vi "TCP Message Interpreter.vi"(8 "error in (no error)":errorcluster, 9 "Data":variant, 10 "Message":string, 11 "Guardian in":refnum<class "Guardian.lvclass">) -> (0 "error out":errorcluster, 3 "Guardian out":refnum<class "Guardian.lvclass">)   [LabVIEW 2020, in "TALOS.lvlib" / "Guardian.lvlib" / "Guardian.lvclass"]
doc: "Use this VI to send a message to the Guardian, from the outside (i.e. from a uService). For internal messages, use the Actor Framework messages system."
uses:
  Guardian.lvclass
  C:/LabVIEW Code/TALOS/builds/Actor Framework PPL/Actor Framework.lvlibp/1abvi3w/vi.lib/ActorFramework/Actor/Actor.lvclass
  C:/LabVIEW Code/TALOS/talos/Ancestor/Ancestor/Ancestor.lvclass
  Ancestor/Ancestor/Ancestor.lvclass/Ancestor.ctl
  Guardian Messages/Ready to launch Msg/Ready to launch Msg.lvclass/Ready to launch Msg.ctl
  Father of all uServices/Father of all uServices/Event Handler Items.ctl
  Guardian.lvclass/Guardian.ctl
  Guardian Messages/Message to uService Msg/Message to uService Msg.lvclass/Message to uService Msg.ctl
  Ancestor/Ancestor/Infinite Message Selector.ctl
  Guardian Messages/Message to Other Guardian Msg/Message to Other Guardian Msg.lvclass/Message to Other Guardian Msg.ctl
  Classes/uService List/uService List.lvclass/uService List.ctl
  Git Update Cluster.ctl
  Abort Message.ctl
  builds/Actor Framework PPL/Actor Framework.lvlibp/1abvi3w/vi.lib/ActorFramework/Message Enqueuer/Message Priority.ctl
  Guardian Messages/Raise or Lower Abort Msg/Raise or Lower Abort Msg.lvclass/Raise or Lower Abort Msg.ctl
  Run Config Data.ctl
  Ancestor/Ancestor/Read Distr uS Map ref.vi
  Ancestor/Ancestor/Write Distr uS Map ref.vi
  Ancestor/Ancestor/Read ID.vi
  Read Guardian List.vi
  Write Guardian List.vi
  FGV/Error Memory/Get Error Description.vi
  Support VIs/Get PC name.vi
  Support VIs/Get Class Name.vi
  <vilib>/Utility/error.llb/Clear Errors.vi
  Support VIs/Circus Root Path.vi
  FGV/Error Memory/Error Memory Core.vi
  <vilib>/AdvancedString/Delimited String to 1D String Array.vi
  FGV/Error Memory/Error Crt Lvl checker.vi
  FGV/Error Memory/Error Memory Core.vi/40c8088d-b597-4017-91af-faa98e00292e.vi
  FGV/Error Memory/Error Memory Core.vi/d4a3ab98-063c-4e44-b43d-fbdcfe6c2be2.vi
  Support VIs/Global Memory.vi
  <vilib>/Utility/LVClass/Get LV Class Name.vi
  Support VIs/TALOS Root path.vi
  Support VIs/Read CSV worksheet.vi
  Support VIs/Global Constants.vi
  <vilib>/Utility/error.llb/General Error Handler.vi
  builds/Actor Framework PPL/Actor Framework.lvlibp/1abvi3w/vi.lib/ActorFramework/Message Enqueuer/Enqueue.vi
  Support VIs/Error Log.vi
  <vilib>/Utility/config.llb/Open Config Data.vi
  <vilib>/Utility/config.llb/Get Section Names.vi
  <vilib>/Utility/config.llb/Get Key Names.vi
  <vilib>/Utility/config.llb/Read Key.vi
  <vilib>/Utility/config.llb/Read Key (String).vi
  <vilib>/Utility/config.llb/Close Config Data.vi
  Ancestor/Ancestor/Ancestor.lvclass
  <vilib>/Comparison/Equal/Equal Functor/Equal Functor.lvclass
  Guardian Messages/Ready to launch Msg/Ready to launch Msg.lvclass
  Guardian Messages/Message to uService Msg/Message to uService Msg.lvclass
  Guardian Messages/Message to Other Guardian Msg/Message to Other Guardian Msg.lvclass
  Classes/Distributed uService Map/Distributed uService Map.lvclass
  Classes/Guardian List/Guardian List.lvclass
  Guardian Messages/Raise or Lower Abort Msg/Raise or Lower Abort Msg.lvclass
  TALOS.lvlib
  Father of all uServices/Father of all uServices/Father of all uServices.lvclass
  builds/Actor Framework PPL/Actor Framework.lvlibp/1abvi3w/vi.lib/ActorFramework/Message Enqueuer/Message Enqueuer.lvclass
  builds/Actor Framework PPL/Actor Framework.lvlibp/1abvi3w/vi.lib/ActorFramework/Actor/Actor.lvclass
  Im alive message.ctl
  Classes/uService List/uService List.lvclass
  Classes/Error Filter/Error Filter.lvclass
  FGV/Error Memory/Error Memory.lvlib
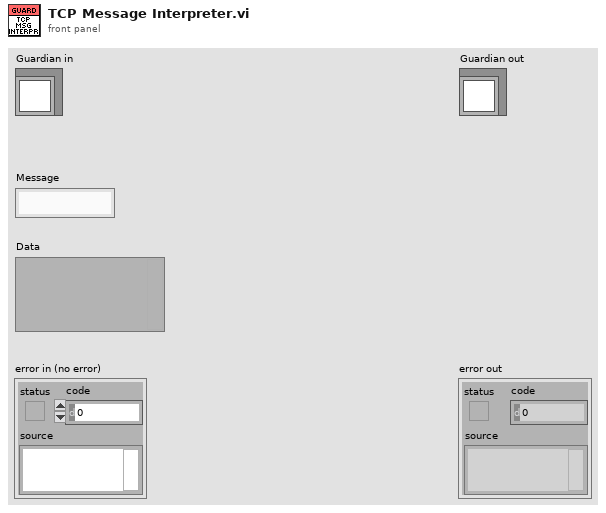
[diagram p1: front panel]
types:
  T1 = typedef "TALOS.lvlib/Father of all uServices.lvlib/Father of all uServices.lvclass/Event Handler Items.ctl" = enum16{"Button Pressed", "Message", "Ready to launch?", "Safe Mode", "Start RUN", "Stop RUN"}
  T2 = typedef "TALOS.lvlib/Ancestor.lvlib/Ancestor.lvclass/Infinite Message Selector.ctl" = enum16{"Start", "Stop", "Check", "Flush (Stop all)", "Init"}
  T3 = typedef "TALOS.lvlib/Guardian.lvlib/Guardian.lvclass/Im alive message.ctl" = cluster{"ID":string, "Time":timestamp, "Abort":bool, "Bearer":bool}
  T4 = typedef "TALOS.lvlib/Guardian.lvlib/Guardian.lvclass/Git Update Cluster.ctl" = cluster{"branch name":string, "include critical PCs":bool, "update from git":bool}
  T5 = typedef "Actor Framework.lvlibp/Message Enqueuer.lvclass/Message Priority.ctl" = enum16{"Low", "Normal", "High"}
  T6 = typedef "TALOS.lvlib/Guardian.lvlib/Guardian.lvclass/Abort Message.ctl" = cluster{"4b0rt":bool, "Sender":string}
  T7 = typedef "TALOS.lvlib/Guardian.lvlib/Guardian.lvclass/Run Config Data.ctl" = cluster{"Name":string, "uS List":string[]}
  T8 = cluster{"Accessors:ID":string, "All IDs":string[]}
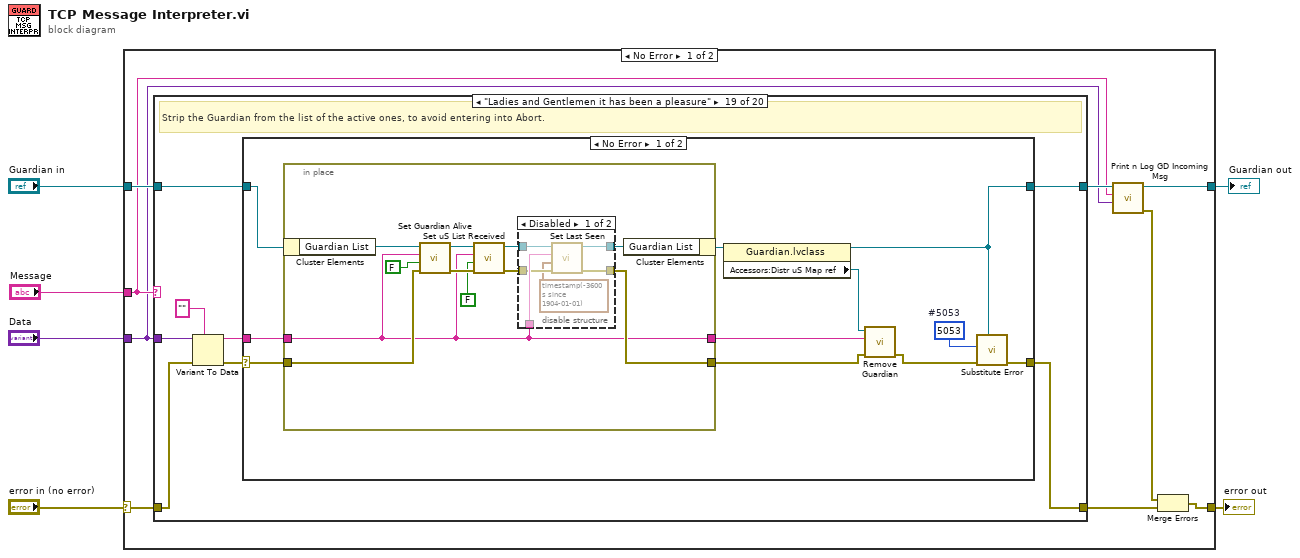
[diagram p0: block diagram]
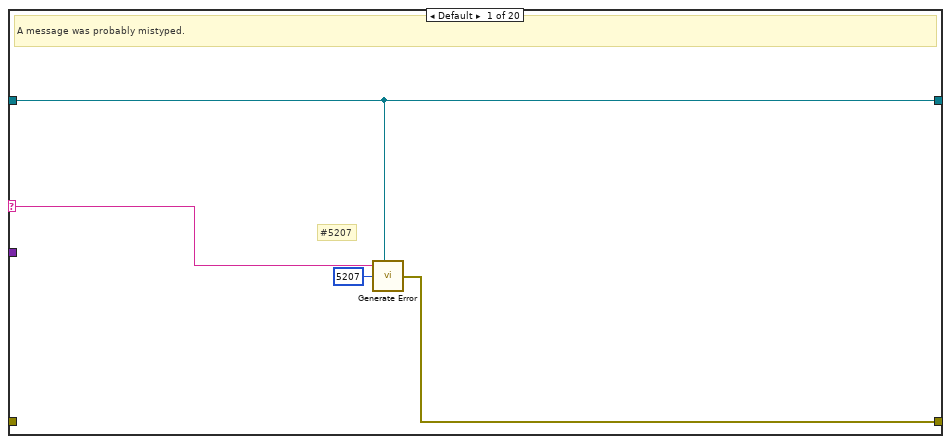
[diagram p2: hidden frame]
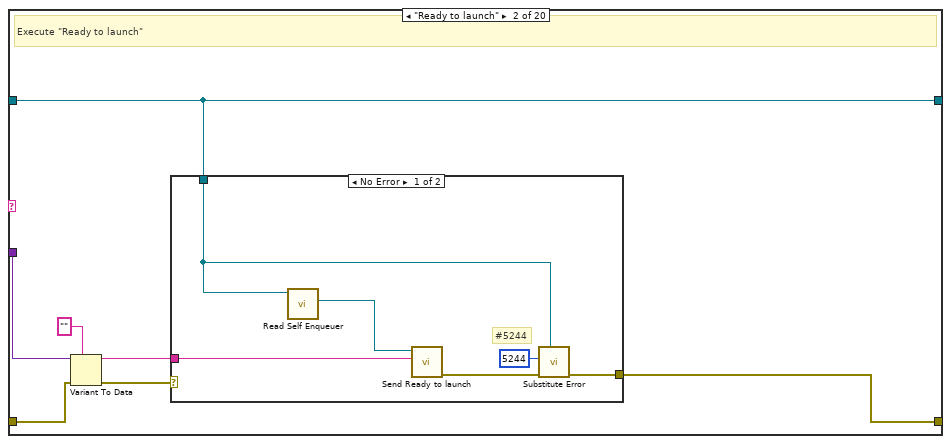
[diagram p3: hidden frame]
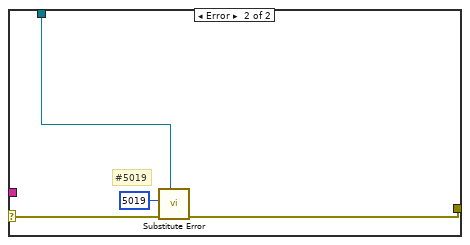
[diagram p4: hidden frame]
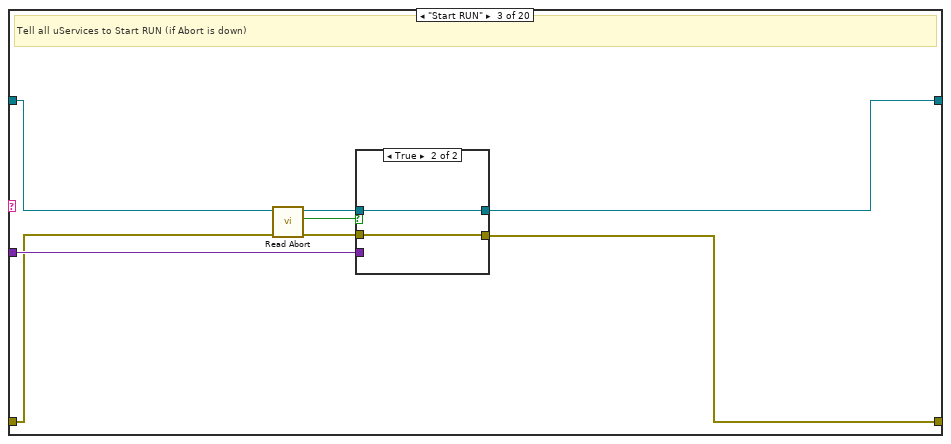
[diagram p5: hidden frame]
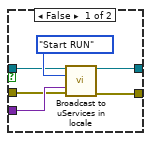
[diagram p6: hidden frame]
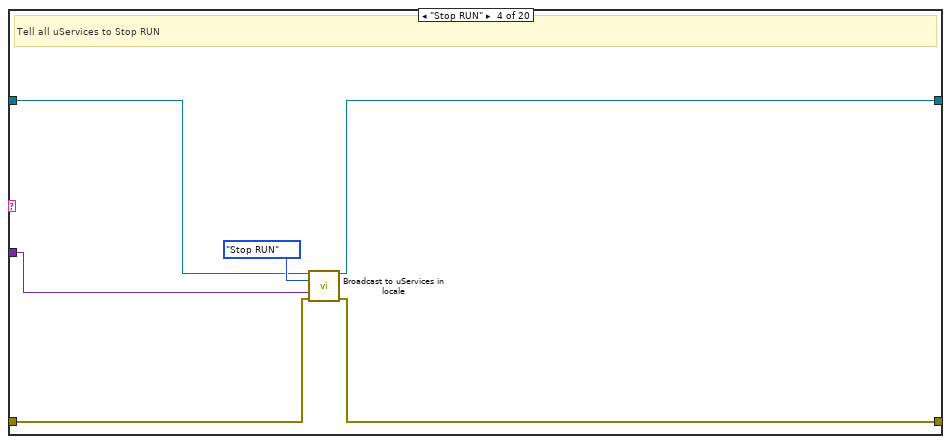
[diagram p7: hidden frame]
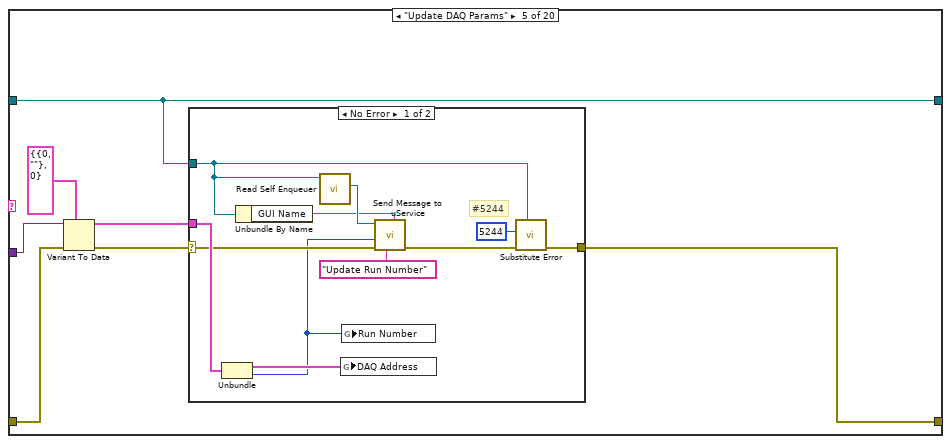
[diagram p8: hidden frame]
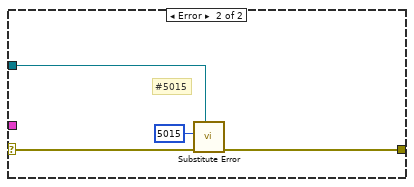
[diagram p9: hidden frame]
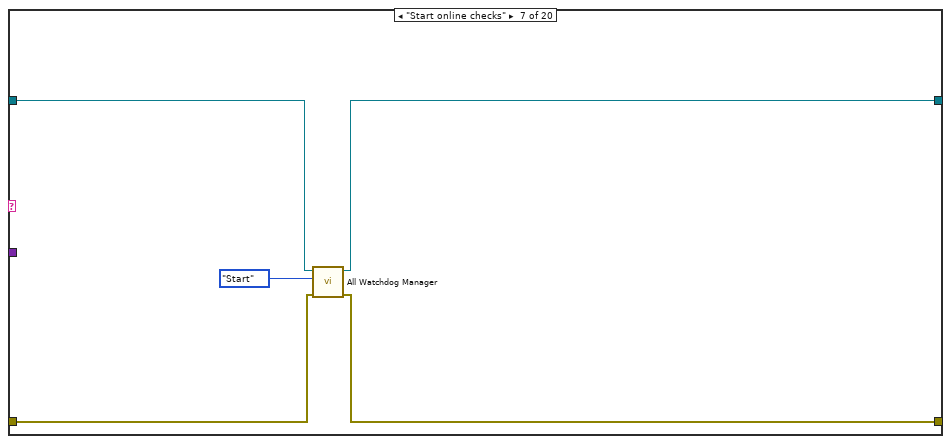
[diagram p11: hidden frame]
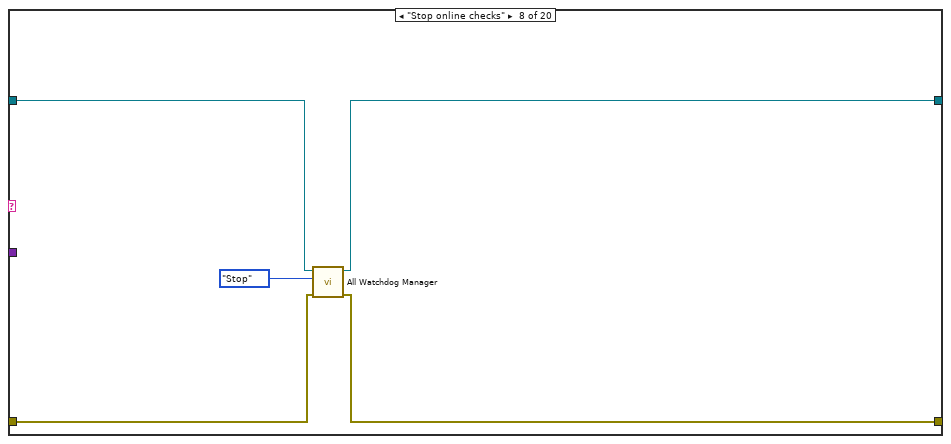
[diagram p12: hidden frame]
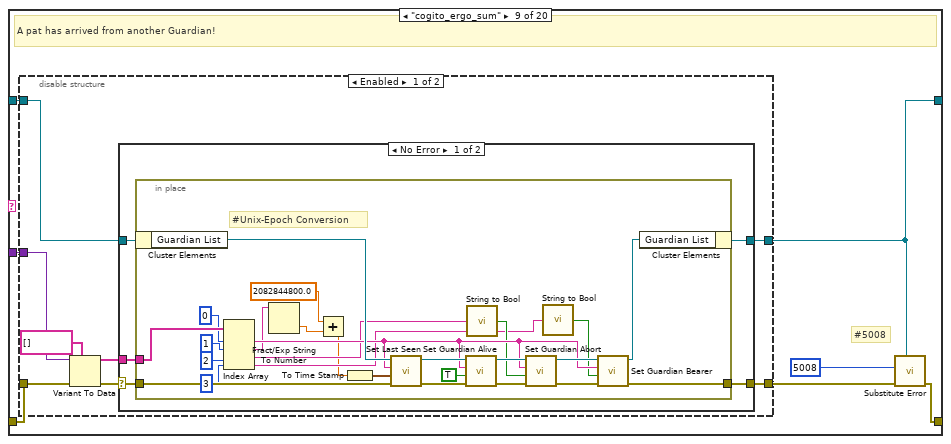
[diagram p13: hidden frame]
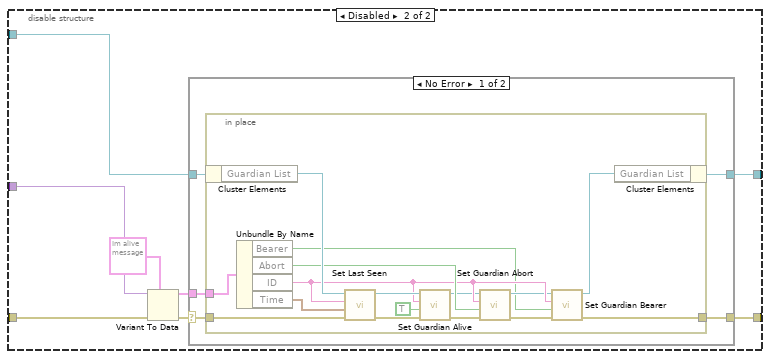
[diagram p15: hidden frame]
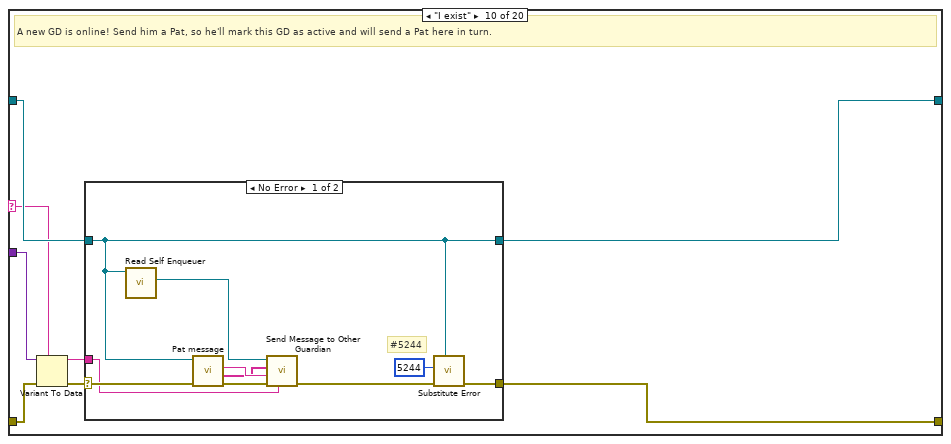
[diagram p17: hidden frame]
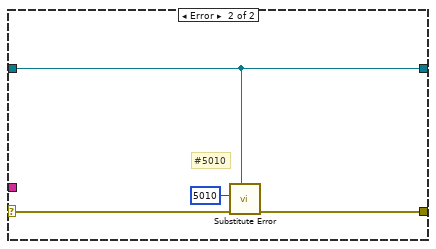
[diagram p18: hidden frame]
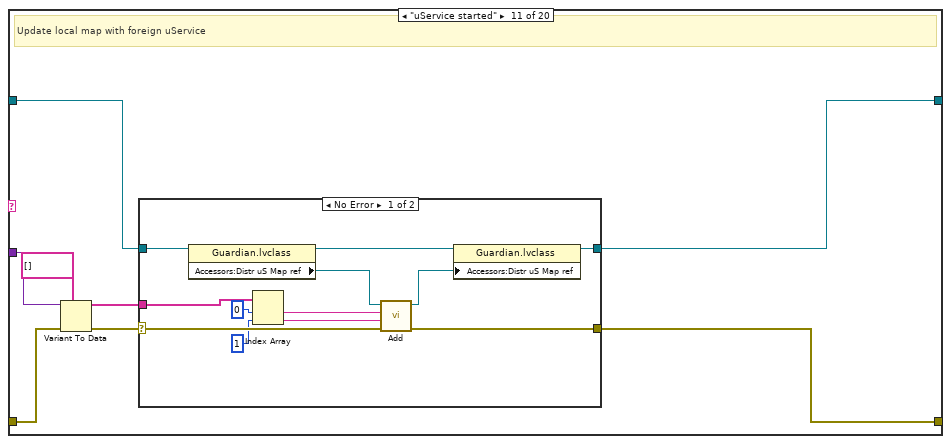
[diagram p19: hidden frame]
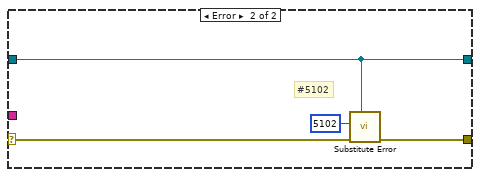
[diagram p20: hidden frame]
diagram:
  n1 = case shown="No Error" "error in (no error)" {
    selector: "error in (no error)" -> [w14 w456]
    tunnel: [w13 w456] -> w6
    tunnel: "Guardian in" -> [w12 w455]
    tunnel: [w10 w455] -> w3
    tunnel: "Data" -> [w8 _]
    tunnel: "Message" -> [w9 _]
    frame No Error {
      n2 = case shown="\"Ladies and Gentlemen it has been a pleasure\"" w9 {
        selector: w9 -> [w17 _ _ _ _ _ _ _ _ w173 _ _ _ _ _ w317 _ _ _ w416]
        tunnel: [w18 w25 w43 w56 w60 w81 w84 w89 w94 w172 w194 w218 w242 w271 w303 w311 w328 w355 w373 w418] -> w15
        tunnel: w8 -> [_ w24 w42 w53 w65 _ _ _ w99 w179 w199 w223 w247 w275 _ w315 w322 w367 w380 w426]
        tunnel: w12 -> [w16 w26 w41 w54 w61 w82 w87 w92 w97 w175 w201 w225 w249 w277 w309 w310 w327 w356 w375 w421]
        tunnel: [w16 w26 w44 w57 w61 w82 w86 w91 w95 w174 w200 w224 w248 w276 w309 w310 w325 w356 w374 w417] -> w11
        tunnel: w14 -> [_ w23 w39 w55 w59 w81 w83 w88 w98 w178 w198 w222 w246 w274 w308 w314 w329 w366 w379 w425]
        frame Default {
          # "#5207"
          # "A message was probably mistyped."
          n3 = call "Generate Error.vi"("Optional String"=w17, "Class"=w16, "Error Code"=5207) -> ("error out"=w18:errorcluster)  [unwired: 4 in]
        }
        frame "Ready to launch" {
          # "Execute \"Ready to launch\""
          n4 = Variant To Data(error in=w23, type="", Variant=w24) -> (data=w20:string, error out=w21:errorcluster)
          n5 = case shown="No Error" w21 {
            selector: w21 -> [_ w35]
            tunnel: w26 -> [w27 w36]
            tunnel: [w28 w34] -> w25
            tunnel: w20 -> [w31 _]
            frame No Error {
              # "#5244"
              n6 = call "Read Self Enqueuer.vi"("Actor"=w27) -> ("Self Enqueuer"=w32:refnum<class "Message Enqueuer.lvclass">)  [unwired: 10 in]
              n7 = call "Send Ready to launch.vi"("GUID"=w31, "Message Enqueuer"=w32) -> ("error out"=w29:errorcluster)  [unwired: 8 in, 1 out]
              n8 = call "Substitute Error.vi"("LabVIEW Object"=w27, "error in (no error)"=w29, "Error Code"=5244) -> ("error out"=w28:errorcluster)  [unwired: 8 in]
            }
            frame Error {
              # "#5019"
              n9 = call "Substitute Error.vi"("LabVIEW Object"=w36, "error in (no error)"=w35, "Error Code"=5019) -> ("error out"=w34:errorcluster)  [unwired: 8 in]
            }
          }
        }
        frame "Start RUN" {
          # "Tell all uServices to Start RUN (if Abort is down)"
          n10 = call "Read Abort.vi"("error in (no error)"=w39, "Guardian in"=w41) -> ("error out"=w38:errorcluster, "Abort"=w37:bool, "Guardian out"=w40:refnum<class "Guardian.lvclass">)  [unwired: 7 in]
          n11 = case shown="True" w37 {
            tunnel: [w49 w52] -> w44
            tunnel: [w48 w51] -> w43
            tunnel: w42 -> [w47 _]
            tunnel: w40 -> [w46 w52]
            tunnel: w38 -> [w45 w51]
            frame False {
              n12 = call "Broadcast to uServices in locale.vi"("Guardian in"=w46, "Event type"=Event_Handler_Items."Start RUN", "Data"=w47, "error in (no error)"=w45) -> ("Guardian out"=w49:refnum<class "Guardian.lvclass">, "error out"=w48:errorcluster)  [unwired: 10 in]
            }
            frame True {
            }
          }
        }
        frame "Stop RUN" {
          # "Tell all uServices to Stop RUN"
          n13 = call "Broadcast to uServices in locale.vi"("Guardian in"=w54, "Event type"=Event_Handler_Items."Stop RUN", "Data"=w53, "error in (no error)"=w55) -> ("Guardian out"=w57:refnum<class "Guardian.lvclass">, "error out"=w56:errorcluster)  [unwired: 10 in]
        }
        frame "Update DAQ Params" {
          n14 = Variant To Data(error in=w59, type=cluster{cluster{u16, string}, i32} {{0, ""}, 0}, Variant=w65) -> (data=w63:cluster{cluster{u16, string}, i32}, error out=w62:errorcluster)
          n15 = case shown="No Error" w62 {
            selector: w62 -> [w73 w80]
            tunnel: w63 -> [w74 _]
            tunnel: w61 -> [w67 w78]
            tunnel: [w66 w79] -> w60
            frame No Error {
              # "#5244"
              n16 = Unbundle(w74) -> (w71:cluster{u16, string}, w70:i32)
              n17 = Unbundle By Name(w67) -> ("GUI Name"=w75:string)
              n18 = call "Read Self Enqueuer.vi"("Actor"=w67) -> ("Self Enqueuer"=w76:refnum<class "Message Enqueuer.lvclass">)  [unwired: 10 in]
              n19 = global write "Global Memory.vi" "DAQ Address"(w71) -> ()
              n20 = global write "Global Memory.vi" "Run Number"(w70) -> ()
              n21 = call "Send Message to uService.vi"("uService ID"=w75, "Message"="Update Run Number", "error in (no error)"=w73, "Data"=w70, "Message Enqueuer"=w76) -> ("error out"=w68:errorcluster)  [unwired: 5 in, 1 out]
              n22 = call "Substitute Error.vi"("LabVIEW Object"=w67, "error in (no error)"=w68, "Error Code"=5244) -> ("error out"=w66:errorcluster)  [unwired: 8 in]
            }
            frame Error {
              # "#5015"
              n23 = call "Substitute Error.vi"("LabVIEW Object"=w78, "error in (no error)"=w80, "Error Code"=5015) -> ("error out"=w79:errorcluster)  [unwired: 8 in]
            }
          }
        }
        frame "Text Message" {
          # "For testing purpouses"
        }
        frame "Start online checks" {
          n24 = call "All Watchdog Manager.vi"("error in (no error)"=w83, "Infinite Message Selector"=Infinite_Message_Selector."Start", "Guardian in"=w87) -> ("error out"=w84:errorcluster, "Guardian out"=w86:refnum<class "Guardian.lvclass">)  [unwired: 6 in, 1 out]
        }
        frame "Stop online checks" {
          n25 = call "All Watchdog Manager.vi"("error in (no error)"=w88, "Infinite Message Selector"=Infinite_Message_Selector."Stop", "Guardian in"=w92) -> ("error out"=w89:errorcluster, "Guardian out"=w91:refnum<class "Guardian.lvclass">)  [unwired: 6 in, 1 out]
        }
        frame "cogito_ergo_sum" {
          # "#5008"
          # "A pat has arrived from another Guardian!"
          n26 = disable-structure shown="Enabled" {
            disable-tunnel: w99 -> [w107 w148]
            disable-tunnel: w98 -> [w106 w146]
            disable-tunnel: w97 -> [w103 w143]
            disable-tunnel: [w102 w142] -> w96
            disable-tunnel: [w101 w141] -> w95
            frame Enabled {
              n27 = Variant To Data(error in=w106, type=string[] [], Variant=w107) -> (data=w105:string[], error out=w104:errorcluster)
              n28 = case shown="No Error" w104 {
                selector: w104 -> [w109 w139]
                tunnel: w105 -> [w110 _]
                tunnel: w103 -> [w112 w140]
                tunnel: [w111 w140] -> w101
                tunnel: [w108 w139] -> w102
                frame No Error {
                  n29 = in-place {
                    in-place-border: w110 -> [w127]
                    in-place-border: w109 -> [w137]
                    in-place-border: [w129] -> w108
                    # "#Unix-Epoch Conversion"
                    n30 = in-place-cluster #1(w112) -> ("Guardian List"=w138:refnum<class "Guardian List.lvclass">)
                    n31 = Index Array(array=w127, index #1=0 ("index"), index #2=1 ("index"), index #3=2 ("index"), index #4=3 ("index")) -> (element #1=w122:string, element #2=w117:string, element #3=w121:string, element #4=w119:string)
                    n32 = Fract/Exp String To Number(string=w117) -> (number=w116:dbl)  [unwired: 3 in, 1 out]
                    n33 = Add(x=2082844800.0, y=w116) -> (x+y=w114:dbl)
                    n34 = To Time Stamp(1:w114) -> (0:w113:timestamp)
                    n35 = call-dynamic "Set Last Seen.vi"("error in (no error)"=w137, "Last Seen"=w113, "ID"=w122, "Guardian List in"=w138) -> ("error out"=w135:errorcluster, "Guardian List out"=w136:refnum<class "Guardian List.lvclass">)  [unwired: 6 in]
                    n36 = call-dynamic "Set Guardian Alive.vi"("error in (no error)"=w135, "Alive"=TRUE, "ID"=w122, "Guardian List in"=w136) -> ("error out"=w133:errorcluster, "Guardian List out"=w128:refnum<class "Guardian List.lvclass">)  [unwired: 6 in]
                    n37 = call "String to Bool.vi"("String"=w121) -> ("Boolean"=w120:bool)
                    n38 = call-dynamic "Set Guardian Abort.vi"("error in (no error)"=w133, "Abort"=w120, "ID"=w122, "Guardian List in"=w128) -> ("error out"=w132:errorcluster, "Guardian List out"=w131:refnum<class "Guardian List.lvclass">)  [unwired: 6 in]
                    n39 = call "String to Bool.vi"("String"=w119) -> ("Boolean"=w118:bool)
                    n40 = call-dynamic "Set Guardian Bearer.vi"("error in (no error)"=w132, "Bearer"=w118, "ID"=w122, "Guardian List in"=w131) -> ("error out"=w129:errorcluster, "Guardian List out"=w130:refnum<class "Guardian List.lvclass">)  [unwired: 6 in]
                    n41 = in-place-cluster #1("Guardian List"=w130) -> (w111:refnum<class "Guardian.lvclass">)
                  }
                }
                frame Error {
                }
              }
            }
            frame Disabled {
              n42 = Variant To Data(error in=w146, type=T3 {"ID"="", "Time"=timestamp(0 s since 1904-01-01), "Abort"=FALSE, "Bearer"=FALSE} ("cluster"), Variant=w148) -> (data=w145:T3, error out=w144:errorcluster)
              n43 = case shown="No Error" w144 {
                selector: w144 -> [w150 w170]
                tunnel: w145 -> [w151 _]
                tunnel: w143 -> [w153 w171]
                tunnel: [w152 w171] -> w141
                tunnel: [w149 w170] -> w142
                frame No Error {
                  n44 = in-place {
                    in-place-border: w151 -> [w168]
                    in-place-border: w150 -> [w166]
                    in-place-border: [w155] -> w149
                    n45 = in-place-cluster #2(w153) -> ("Guardian List"=w169:refnum<class "Guardian List.lvclass">)
                    n46 = Unbundle By Name(w168) -> ("Bearer"=w157:bool, "Abort"=w160:bool, "ID"=w159:string, "Time"=w167:timestamp)
                    n47 = call-dynamic "Set Last Seen.vi"("error in (no error)"=w166, "Last Seen"=w167, "ID"=w159, "Guardian List in"=w169) -> ("error out"=w164:errorcluster, "Guardian List out"=w165:refnum<class "Guardian List.lvclass">)  [unwired: 6 in]
                    n48 = call-dynamic "Set Guardian Alive.vi"("error in (no error)"=w164, "Alive"=TRUE, "ID"=w159, "Guardian List in"=w165) -> ("error out"=w162:errorcluster, "Guardian List out"=w154:refnum<class "Guardian List.lvclass">)  [unwired: 6 in]
                    n49 = call-dynamic "Set Guardian Abort.vi"("error in (no error)"=w162, "Abort"=w160, "ID"=w159, "Guardian List in"=w154) -> ("error out"=w161:errorcluster, "Guardian List out"=w158:refnum<class "Guardian List.lvclass">)  [unwired: 6 in]
                    n50 = call-dynamic "Set Guardian Bearer.vi"("error in (no error)"=w161, "Bearer"=w157, "ID"=w159, "Guardian List in"=w158) -> ("error out"=w155:errorcluster, "Guardian List out"=w156:refnum<class "Guardian List.lvclass">)  [unwired: 6 in]
                    n51 = in-place-cluster #2("Guardian List"=w156) -> (w152:refnum<class "Guardian.lvclass">)
                  }
                }
                frame Error {
                }
              }
            }
          }
          n52 = call "Substitute Error.vi"("LabVIEW Object"=w95, "error in (no error)"=w96, "Error Code"=5008) -> ("error out"=w94:errorcluster)  [unwired: 8 in]
        }
        frame "I exist" {
          # "A new GD is online! Send him a Pat, so he'll mark this GD as active and will send a Pat here in turn."
          n53 = Variant To Data(error in=w178, type=w173, Variant=w179) -> (data=w177:string, error out=w176:errorcluster)
          n54 = case shown="No Error" w176 {
            selector: w176 -> [w188 w192]
            tunnel: w177 -> [w187 _]
            tunnel: w175 -> [w181 w193]
            tunnel: [w181 w193] -> w174
            tunnel: [w180 w190] -> w172
            frame No Error {
              # "#5244"
              n55 = call "Read Self Enqueuer.vi"("Actor"=w181) -> ("Self Enqueuer"=w189:refnum<class "Message Enqueuer.lvclass">)  [unwired: 10 in]
              n56 = call "Pat message.vi"("error in (no error)"=w188, "Guardian in"=w181) -> ("error out"=w184:errorcluster, "Data"=w185:string[], "Message name"=w186:string)  [unwired: 6 in, 1 out]
              n57 = call "Send Message to Other Guardian.vi"("Guardian ID"=w187, "error in (no error)"=w184, "Message"=w186, "Data"=w185, "Message Enqueuer"=w189) -> ("error out"=w182:errorcluster)  [unwired: 5 in, 1 out]
              n58 = call "Substitute Error.vi"("LabVIEW Object"=w181, "error in (no error)"=w182, "Error Code"=5244) -> ("error out"=w180:errorcluster)  [unwired: 8 in]
            }
            frame Error {
              # "#5010"
              n59 = call "Substitute Error.vi"("LabVIEW Object"=w193, "error in (no error)"=w192, "Error Code"=5010) -> ("error out"=w190:errorcluster)  [unwired: 8 in]
            }
          }
        }
        frame "uService started" {
          # "Update local map with foreign uService"
          n60 = Variant To Data(error in=w198, type=string[] [], Variant=w199) -> (data=w195:string[], error out=w196:errorcluster)
          n61 = case shown="No Error" w196 {
            selector: w196 -> [w213 w217]
            tunnel: w201 -> [w206 w215]
            tunnel: [w203 w215] -> w200
            tunnel: w195 -> [w211 _]
            tunnel: [w212 w214] -> w194
            frame No Error {
              n62 = property class="Guardian.lvclass"(reference=w206) -> (reference out=w204:refnum<class "Guardian.lvclass">, "Accessors:Distr uS Map ref"=w205:refnum<data-value>)  [unwired: 1 in, 1 out]
              n63 = Index Array(array=w211, index #1=0 ("index"), index #2=1 ("index")) -> (element #1=w208:string, element #2=w207:string)
              n64 = call "Add.vi"("error in (no error)"=w213, "uService"=w207, "Guardian"=w208, "Distr uS Map ref in"=w205) -> ("error out"=w212:errorcluster, "Distr uS Map ref out"=w202:refnum<data-value>)  [unwired: 5 in, 1 out]
              n65 = property class="Guardian.lvclass"(reference=w204, "Accessors:Distr uS Map ref"=w202) -> (reference out=w203:refnum<class "Guardian.lvclass">)  [unwired: 1 in, 1 out]
            }
            frame Error {
              # "#5102"
              n66 = call "Substitute Error.vi"("LabVIEW Object"=w215, "error in (no error)"=w217, "Error Code"=5102) -> ("error out"=w214:errorcluster)  [unwired: 8 in]
            }
          }
        }
        frame "uService stopped" {
          # "Update local map with foreign uService"
          n67 = Variant To Data(error in=w222, type=string[] [], Variant=w223) -> (data=w219:string[], error out=w220:errorcluster)
          n68 = case shown="No Error" w220 {
            selector: w220 -> [w236 w241]
            tunnel: w225 -> [w237 w239]
            tunnel: [w227 w239] -> w224
            tunnel: w219 -> [w234 _]
            tunnel: [w235 w238] -> w218
            frame No Error {
              n69 = property class="Guardian.lvclass"(reference=w237) -> (reference out=w228:refnum<class "Guardian.lvclass">, "Accessors:Distr uS Map ref"=w229:refnum<data-value>)  [unwired: 1 in, 1 out]
              n70 = Index Array(array=w234, index #1=0 ("index"), index #2=1 ("index")) -> (element #1=w231:string, element #2=w230:string)
              n71 = call "Remove.vi"("error in (no error)"=w236, "uService ID"=w230, "Guardian"=w231, "Distr uS Map ref in"=w229) -> ("error out"=w235:errorcluster, "Distr uS Map ref out"=w226:refnum<data-value>)  [unwired: 5 in, 1 out]
              n72 = property class="Guardian.lvclass"(reference=w228, "Accessors:Distr uS Map ref"=w226) -> (reference out=w227:refnum<class "Guardian.lvclass">)  [unwired: 1 in, 1 out]
            }
            frame Error {
              # "#5102"
              n73 = call "Substitute Error.vi"("LabVIEW Object"=w239, "error in (no error)"=w241, "Error Code"=5102) -> ("error out"=w238:errorcluster)  [unwired: 8 in]
            }
          }
        }
        frame "Get uService List" {
          # "Give to the requesting Guardian the current uService List (for initialise the distributed one)"
          n74 = Variant To Data(error in=w246, type="", Variant=w247) -> (data=w243:string, error out=w244:errorcluster)
          n75 = case shown="No Error" w244 {
            selector: w244 -> [w260 w269]
            tunnel: w249 -> [w261 w267]
            tunnel: [w250 w267] -> w248
            tunnel: w243 -> [w265 _]
            tunnel: [w251 w266] -> w242
            frame No Error {
              # "#5244"
              # "requesting GD"
              n76 = call-dynamic "Access uService List.vi"("error in (no error)"=w260, "Ancestor in"=w261) -> ("error out"=w258:errorcluster, "uService List out"=w259:refnum<class "uService List.lvclass">, "Ancestor out"=w262:refnum<class "Guardian.lvclass">)  [unwired: 7 in]
              n77 = call "Get all IDs.vi"("error in (no error)"=w258, "uService List"=w259) -> ("error out"=w257:errorcluster, "All IDs"=w255:string[])  [unwired: 7 in, 1 out]
              n78 = property class="Guardian.lvclass"(reference=w262) -> (reference out=w250:refnum<class "Guardian.lvclass">, "Accessors:ID"=w256:string)  [unwired: 1 in, 1 out]
              n79 = Bundle("Accessors:ID"=w256, "All IDs"=w255) -> (w254:T8)  [unwired: 1 in]
              n80 = call "Read Self Enqueuer.vi"("Actor"=w250) -> ("Self Enqueuer"=w264:refnum<class "Message Enqueuer.lvclass">)  [unwired: 10 in]
              n81 = call "Send Message to Other Guardian.vi"("Guardian ID"=w265, "error in (no error)"=w257, "Message"="Current uService List", "Data"=w254, "Message Enqueuer"=w264) -> ("error out"=w252:errorcluster)  [unwired: 5 in, 1 out]
              n82 = call "Substitute Error.vi"("LabVIEW Object"=w250, "error in (no error)"=w252, "Error Code"=5244) -> ("error out"=w251:errorcluster)  [unwired: 8 in]
            }
            frame Error {
              # "#5102"
              n83 = call "Substitute Error.vi"("LabVIEW Object"=w267, "error in (no error)"=w269, "Error Code"=5102) -> ("error out"=w266:errorcluster)  [unwired: 8 in]
            }
          }
        }
        frame "Current uService List" {
          # "Update Distributed uService List with the list received"
          n84 = Variant To Data(error in=w274, type=cluster{"String":string, string[]} {"String"="", []}, Variant=w275) -> (data=w272:cluster{"String":string, string[]}, error out=w273:errorcluster)
          n85 = case shown="No Error" w273 {
            selector: w273 -> [w291 w302]
            tunnel: w277 -> [w284 w300]
            tunnel: [w283 w300] -> w276
            tunnel: w272 -> [w292 _]
            tunnel: [w290 w299] -> w271
            frame No Error {
              n86 = property class="Guardian.lvclass"(reference=w284) -> (reference out=w280:refnum<class "Guardian.lvclass">, "Accessors:Distr uS Map ref"=w279:refnum<data-value>, "Accessors:Guardian List"=w278:refnum<class "Guardian List.lvclass">)  [unwired: 1 in, 1 out]
              n87 = Unbundle(w292) -> ("String"=w287:string, w289:string[])
              n88 = for {
                shift-right: [w294] -> w282
                shift-left: w279 -> [w293]
                tunnel: w287 -> [w298]
                tunnel: w289 -> [w297] mode=indexing
                shift-right: [w295] -> w288
                shift-left: w291 -> [w296]
                n89 = call "Add.vi"("error in (no error)"=w296, "uService"=w297, "Guardian"=w298, "Distr uS Map ref in"=w293) -> ("error out"=w295:errorcluster, "Distr uS Map ref out"=w294:refnum<data-value>)  [unwired: 5 in, 1 out]
              }
              n90 = call-dynamic "Set uS List Received.vi"("uS List Received"=TRUE, "ID"=w287, "Guardian List in"=w278) -> ("error out"=w286:errorcluster, "Guardian List out"=w281:refnum<class "Guardian List.lvclass">)  [unwired: 7 in]
              n91 = Merge Errors(w288, w286) -> (w290:errorcluster)
              n92 = property class="Guardian.lvclass"(reference=w280, "Accessors:Distr uS Map ref"=w282, "Accessors:Guardian List"=w281) -> (reference out=w283:refnum<class "Guardian.lvclass">)  [unwired: 1 in, 1 out]
            }
            frame Error {
              # "#5102"
              n93 = call "Substitute Error.vi"("LabVIEW Object"=w300, "error in (no error)"=w302, "Error Code"=5102) -> ("error out"=w299:errorcluster)  [unwired: 8 in]
            }
          }
        }
        frame "Reload INI files" {
          w306 = TRUE ("Load")
          # "Reload the configuration files"
          n94 = call "TALOS Config Param.vi"("Load"=w306, "error in (no error)"=w308) -> ("error out"=w307:errorcluster)  [unwired: 8 in, 1 out]
          n95 = call "Circus Config Param - Core.vi"("Load"=w306, "error in (no error)"=w307) -> ("error out"=w305:errorcluster)  [unwired: 8 in, 1 out]
          n96 = call "Errors Load.vi"("error in (no error)"=w305) -> ("error out"=w304:errorcluster)  [unwired: 10 in]
          n97 = call "Init.vi"("error in (no error)"=w304) -> ("error out"=w303:errorcluster)  [unwired: 10 in]
        }
        frame "Change Run LED color", "Reset Run LED", "Run Stopped with Errors", "Update Error Listbox", "Update Kasli Log", "Update Run Status" {
          # "#5244"
          n98 = Unbundle By Name(w310) -> ("GUI Name"=w318:string)
          n99 = call "Read Self Enqueuer.vi"("Actor"=w310) -> ("Self Enqueuer"=w319:refnum<class "Message Enqueuer.lvclass">)  [unwired: 10 in]
          n100 = call "Send Message to uService.vi"("uService ID"=w318, "Message"=w317, "error in (no error)"=w314, "Data"=w315, "Locale?"=TRUE, "Message Enqueuer"=w319) -> ("error out"=w312:errorcluster)  [unwired: 4 in, 1 out]
          n101 = call "Substitute Error.vi"("LabVIEW Object"=w310, "error in (no error)"=w312, "Error Code"=5244) -> ("error out"=w311:errorcluster)  [unwired: 8 in]
        }
        frame "Update from GIT" {
          n102 = Variant To Data(type=T4 {"branch name"="", "include critical PCs"=FALSE, "update from git"=FALSE} ("Git update cluster"), Variant=w322) -> (data=w320:T4)  [unwired: 1 in, 1 out]
          n103 = flat-sequence {
            tunnel: w329 -> [_]
            tunnel: [w330] -> w323
            tunnel: w327 -> [w338]
            tunnel: [w337] -> w324
            tunnel: w320 -> [w336]
            tunnel: w327 -> [w354]
            tunnel: [w353] -> w326
            tunnel: [w352] -> w325
            frame #0 {
              n104 = for {
                tunnel: i32[] [5004, 5005] ("Error Code") -> [w333] mode=indexing
                tunnel: [w332] -> w330 mode=indexing
                n105 = call "Add.vi"("Error Code"=w333) -> ("error out"=w332:errorcluster)  [unwired: 10 in]
              }
            }
            frame #1 {
              n106 = global read "Global Constants.vi" "Local"() -> (w342:bool)
              n107 = call "Is in Packed Library.vi"() -> ("error out"=w343:errorcluster, "Is In Packed Library"=w340:bool)  [unwired: 10 in]
              n108 = Unbundle By Name(w336) -> ("update from git"=w335:bool, "branch name"=w334:string)
              n109 = Not(x=w340) -> (.not. x?=w341:bool)
              n110 = Or(x=w342, y=w341) -> (x .or. y?=w339:bool)
              n111 = case shown="False" w339 {
                tunnel: w343 -> [w348 w351]
                tunnel: [w347 w350] -> w337
                tunnel: w338 -> [w346 _]
                tunnel: w335 -> [w345 _]
                tunnel: w334 -> [w344 _]
                frame False {
                  n112 = call "Launch Update from Git.vi"("error in (no error)"=w348, "Branch name"=w344, "Update GIT"=w345, "Guardian in"=w346) -> ("error out"=w347:errorcluster)  [unwired: 6 in, 1 out]
                }
                frame True {
                  n113 = call "Temporised Pop-up Window.vi"("error in (no error)"=w351, "Text"="I'm dying!") -> ("error out"=w350:errorcluster)  [unwired: 9 in]
                }
              }
            }
            frame #2 {
              n114 = call "System shutdown.vi"("Guardian in"=w354) -> ("error out"=w353:errorcluster, "Guardian out"=w352:refnum<class "Guardian.lvclass">)  [unwired: 9 in]
            }
          }
          n115 = Merge Errors(w326, w324, w323) -> (w328:errorcluster)
        }
        frame "4b0rt" {
          # "#5244"
          # "I don't throw an error here because it will likely cause a loop"
          # "Directly run the \"Raise/Lower Abort\" VI creates a recursive loop, so need ot call it as a message."
          n116 = Variant To Data(error in=w366, type=T6 {"4b0rt"=FALSE, "Sender"=""} ("4b0rt Message"), Variant=w367) -> (data=w363:T6, error out=w364:errorcluster)
          n117 = case shown="No Error" w364 {
            tunnel: w363 -> [w370 _]
            tunnel: [w369 "local" ("Sender")] -> w362
            tunnel: [w368 TRUE ("New Abort Value")] -> w361
            frame No Error {
              n118 = Unbundle By Name(w370) -> ("4b0rt"=w368:bool, "Sender"=w369:string)
            }
            frame Error {
            }
          }
          n119 = call "Read Self Enqueuer.vi"("Actor"=w356) -> ("Self Enqueuer"=w360:refnum<class "Message Enqueuer.lvclass">)  [unwired: 10 in]
          n120 = call "Send Raise or Lower Abort.vi"("Message Priority (Normal)"=Message_Priority."High", "Sender"=w362, "New Abort Value"=w361, "Message Enqueuer"=w360) -> ("error out"=w357:errorcluster)  [unwired: 6 in, 1 out]
          n121 = call "Substitute Error.vi"("LabVIEW Object"=w356, "error in (no error)"=w357, "Error Code"=5244) -> ("error out"=w355:errorcluster)  [unwired: 8 in]
        }
        frame "Ladies and Gentlemen it has been a pleasure" {
          # "Strip the Guardian from the list of the active ones, to avoid entering into Abort."
          n122 = Variant To Data(error in=w379, type="", Variant=w380) -> (data=w376:string, error out=w377:errorcluster)
          n123 = case shown="No Error" w377 {
            selector: w377 -> [w389 w415]
            tunnel: w376 -> [w390 w412]
            tunnel: w375 -> [w391 w413]
            tunnel: [w385 w413] -> w374
            tunnel: [w387 w411] -> w373
            frame No Error {
              w388 = 5053  # #5053
              n124 = in-place {
                in-place-border: w390 -> [w393]
                in-place-border: w389 -> [w400]
                in-place-border: [w398] -> w382
                in-place-border: [w393] -> w383
                n125 = in-place-cluster #3(w391) -> ("Guardian List"=w402:refnum<class "Guardian List.lvclass">)
                n126 = call-dynamic "Set Guardian Alive.vi"("error in (no error)"=w400, "Alive"=FALSE, "ID"=w393, "Guardian List in"=w402) -> ("error out"=w394:errorcluster, "Guardian List out"=w397:refnum<class "Guardian List.lvclass">)  [unwired: 6 in]
                n127 = call-dynamic "Set uS List Received.vi"("error in (no error)"=w394, "uS List Received"=FALSE, "ID"=w393, "Guardian List in"=w397) -> ("error out"=w395:errorcluster, "Guardian List out"=w396:refnum<class "Guardian List.lvclass">)  [unwired: 6 in]
                n128 = disable-structure shown="Disabled" {
                  disable-tunnel: w396 -> [w408 w410]
                  disable-tunnel: [w407 w410] -> w401
                  disable-tunnel: w393 -> [w406 _]
                  disable-tunnel: w395 -> [w405 w409]
                  disable-tunnel: [w403 w409] -> w398
                  frame Disabled {
                    n129 = call-dynamic "Set Last Seen.vi"("error in (no error)"=w405, "Last Seen"=timestamp(-3600 s since 1904-01-01) ("y"), "ID"=w406, "Guardian List in"=w408) -> ("error out"=w403:errorcluster, "Guardian List out"=w407:refnum<class "Guardian List.lvclass">)  [unwired: 6 in]
                  }
                  frame Enabled {
                  }
                }
                n130 = in-place-cluster #3("Guardian List"=w401) -> (w386:refnum<class "Guardian.lvclass">)
              }
              n131 = property class="Guardian.lvclass"(reference=w386) -> (reference out=w385:refnum<class "Guardian.lvclass">, "Accessors:Distr uS Map ref"=w384:refnum<data-value>)  [unwired: 1 in, 1 out]
              n132 = call "Remove Guardian.vi"("error in (no error)"=w382, "Guardian ID"=w383, "Distr uS Map ref in"=w384) -> ("error out"=w381:errorcluster)  [unwired: 7 in, 1 out]
              n133 = call "Substitute Error.vi"("LabVIEW Object"=w385, "error in (no error)"=w381, "Error Code"=w388) -> ("error out"=w387:errorcluster)  [unwired: 8 in]
            }
            frame Error {
              w414 = 5207  # #5207
              n134 = call "Substitute Error.vi"("LabVIEW Object"=w413, "error in (no error)"=w415, "Error Code"=w414, "Optional String"=w412) -> ("error out"=w411:errorcluster)  [unwired: 7 in]
            }
          }
        }
        frame "Add uSs from Config", "Change Run Config", "Realign uSs from Config" {
          w420 = 5056  # #5056
          # "Load the new Run Config file, stop and launch uServices accordingly."
          n135 = Variant To Data(error in=w425, type=T7 {"Name"="", "uS List"=[]} ("Run Config Data"), Variant=w426) -> (data=w422:T7, error out=w423:errorcluster)
          n136 = case shown="No Error" w423 {
            selector: w423 -> [w435 w454]
            tunnel: w422 -> [w436 _]
            tunnel: w421 -> [w437 w453]
            tunnel: [w427 w454] -> w419
            tunnel: [w428 w453] -> w417
            tunnel: w416 -> [w432 _]
            frame No Error {
              n137 = Unbundle By Name(w436) -> ("Name"=w434:string, "uS List"=w430:string[])
              n138 = Unbundle By Name(w437) -> ("GUI Name"=w439:string)
              n139 = call "Read Self Enqueuer.vi"("Actor"=w437) -> ("Self Enqueuer"=w440:refnum<class "Message Enqueuer.lvclass">)  [unwired: 10 in]
              n140 = Bundle By Name(cluster=w437, "Run Config Data"=w436) -> (w429:refnum<class "Guardian.lvclass">)
              n141 = call "Send Message to uService.vi"("uService ID"=w439, "Message"="Update Run Config", "error in (no error)"=w435, "Data"=w434, "Locale?"=TRUE, "Message Enqueuer"=w440) -> ("error out"=w431:errorcluster)  [unwired: 4 in, 1 out]
              n142 = case shown="\"Realign uSs from Config\"" w432 {
                tunnel: w431 -> [w441 w447 w452]
                tunnel: w430 -> [_ w446 w450]
                tunnel: w429 -> [w442 w445 w449]
                tunnel: [w442 w444 w448] -> w428
                tunnel: [w441 w443 w451] -> w427
                frame "Change Run Config", Default {
                  # "Do nothing on uSs."
                }
                frame "Add uSs from Config" {
                  n143 = call "Add uSs from Run Config.vi"("error in (no error)"=w447, "uS List"=w446, "Guardian in"=w445) -> ("error out"=w443:errorcluster, "Guardian out"=w444:refnum<class "Guardian.lvclass">)  [unwired: 7 in]
                }
                frame "Realign uSs from Config" {
                  n144 = call "Realign uSs from Run Config.vi"("error in (no error)"=w452, "uS List"=w450, "Guardian in"=w449) -> ("error out"=w451:errorcluster, "Guardian out"=w448:refnum<class "Guardian.lvclass">)  [unwired: 7 in]
                }
              }
            }
            frame Error {
            }
          }
          n145 = call "Substitute Error.vi"("LabVIEW Object"=w417, "error in (no error)"=w419, "Error Code"=w420) -> ("error out"=w418:errorcluster)  [unwired: 8 in]
        }
      }
      n146 = call "Print n Log GD Incoming Msg.vi"("Data"=w8, "Message"=w9, "Guardian in"=w11) -> ("error out"=w7:errorcluster, "Guardian out"=w10:refnum<class "Guardian.lvclass">)  [unwired: 7 in]
      n147 = Merge Errors(w7, w15) -> (w13:errorcluster)
    }
    frame Error {
    }
  }
  "error out" <- w6
  "Guardian out" <- w3
